vi "Login.vi"(8 "error in (no error) 3":errorcluster) -> (0 "error in (no error) 4":errorcluster, 3 "Enum":T2)   [LabVIEW 2021]
uses:
  Control/login_type.ctl
  Control/User_login_type.ctl
  Control/add_remove.ctl
  Template/Main_VI/Control/Ini.ctl
panel:
  in  "USER TYPE":T1 items=["Admin", "Operator"]
  out "element 3":string
  out "Array 2":string[](array[string])
  in  "PASSWORD":string
  in  "NAME":T1
  out "element 2":string
  in  "Remove user":bool
  out "Boolean 4":bool=TRUE
  out "Numeric":i32
  out "Boolean 3":bool=TRUE
  in  "Back Button":bool
  in  "Enum":T2
  in  "error in (no error) 2":errorcluster
  out "error out":errorcluster
  out "Result":bool
  out "element":string
  out "Ring - Menu 2":u16(ring)
  in  "error in (no error)":errorcluster
  out "array w/ subset deleted":string[](array[string])
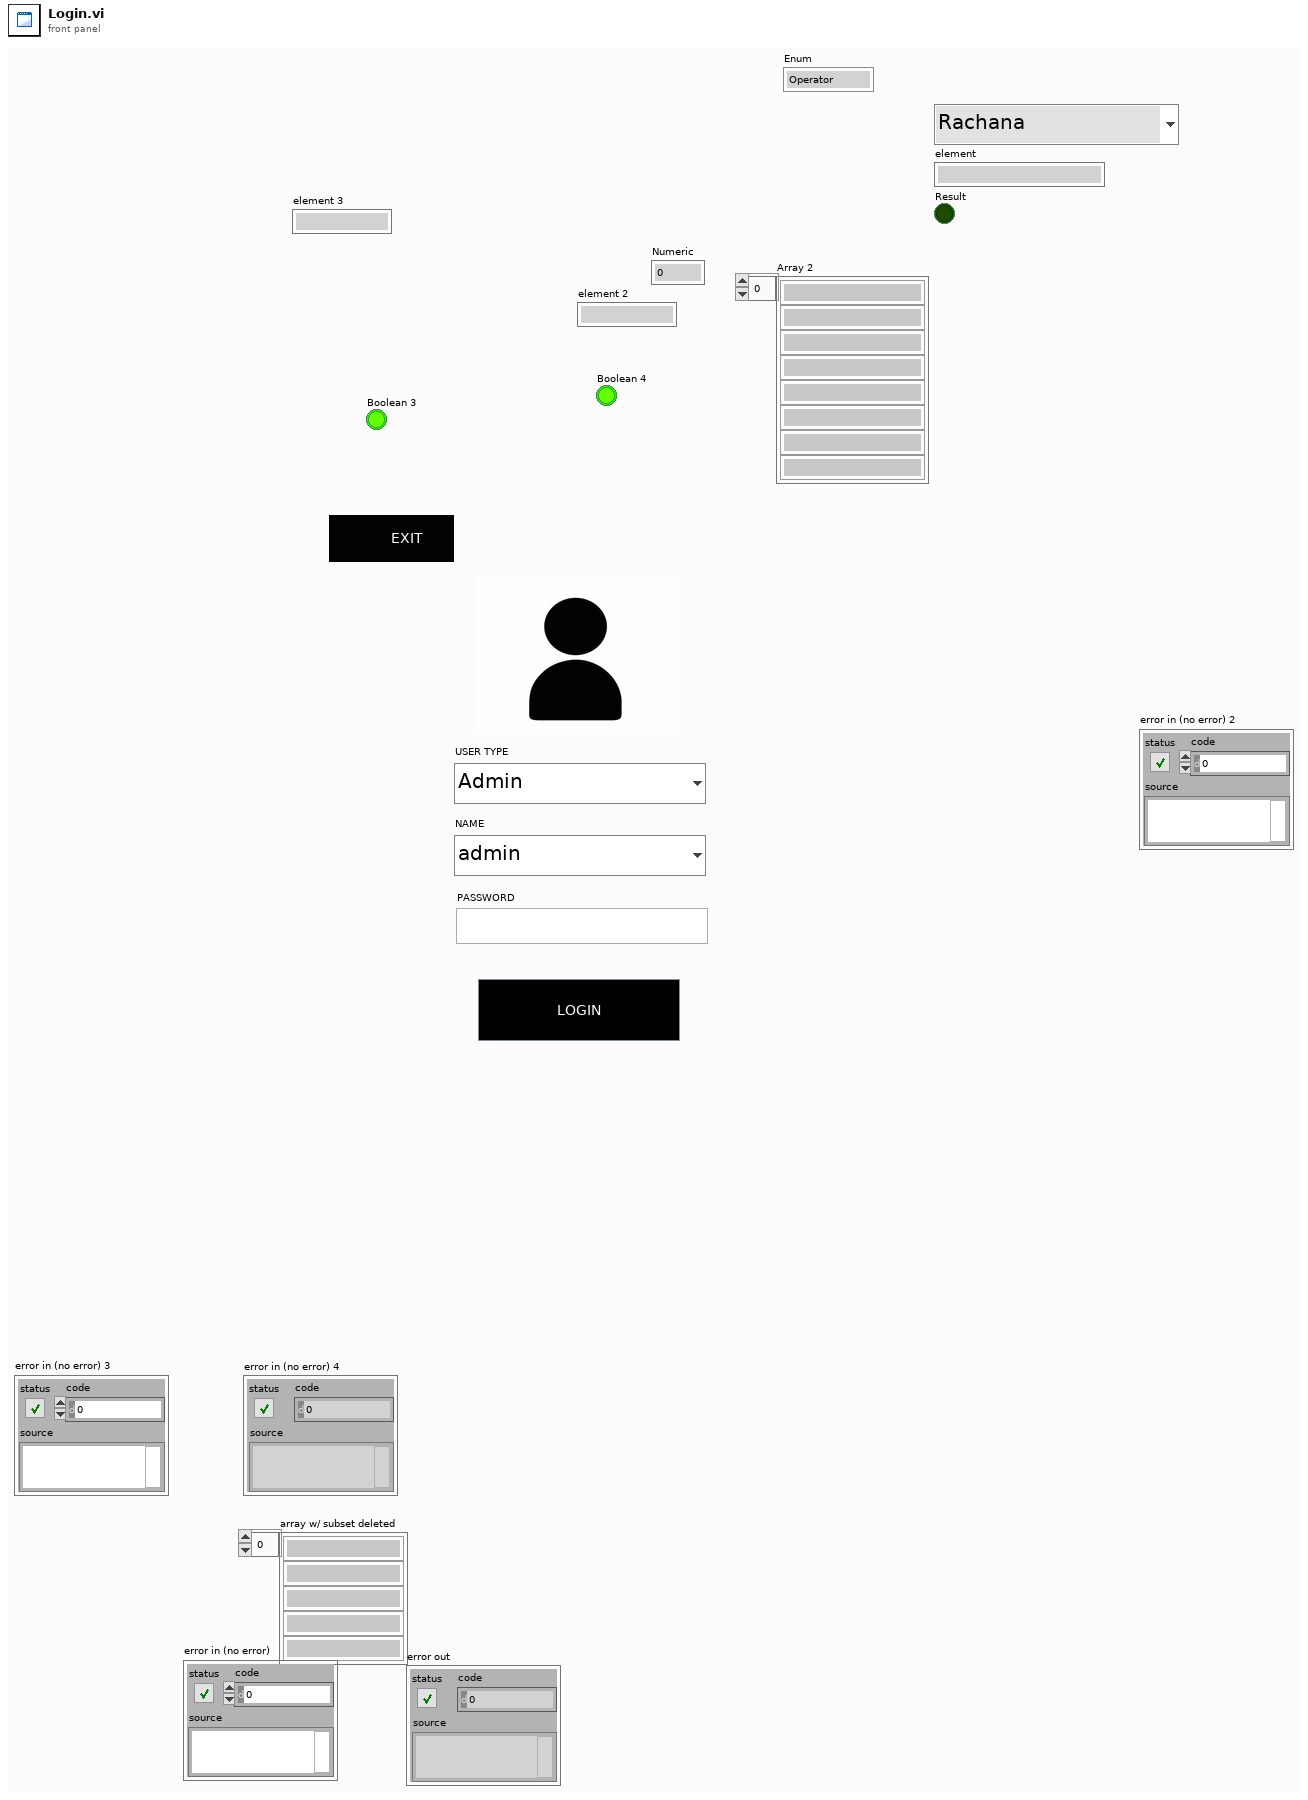
[diagram p1: front panel]
types:
  T1 = typedef "User_login_type.ctl" = u16
  T2 = typedef "login_type.ctl" = enum16{"Operator", "Admin"}
  T3 = typedef "add_remove.ctl" = enum16{"Enter", "add user", "remover user", "view user"}
  T4 = typedef "Ini.ctl" = enum16{"Write", "Read"}
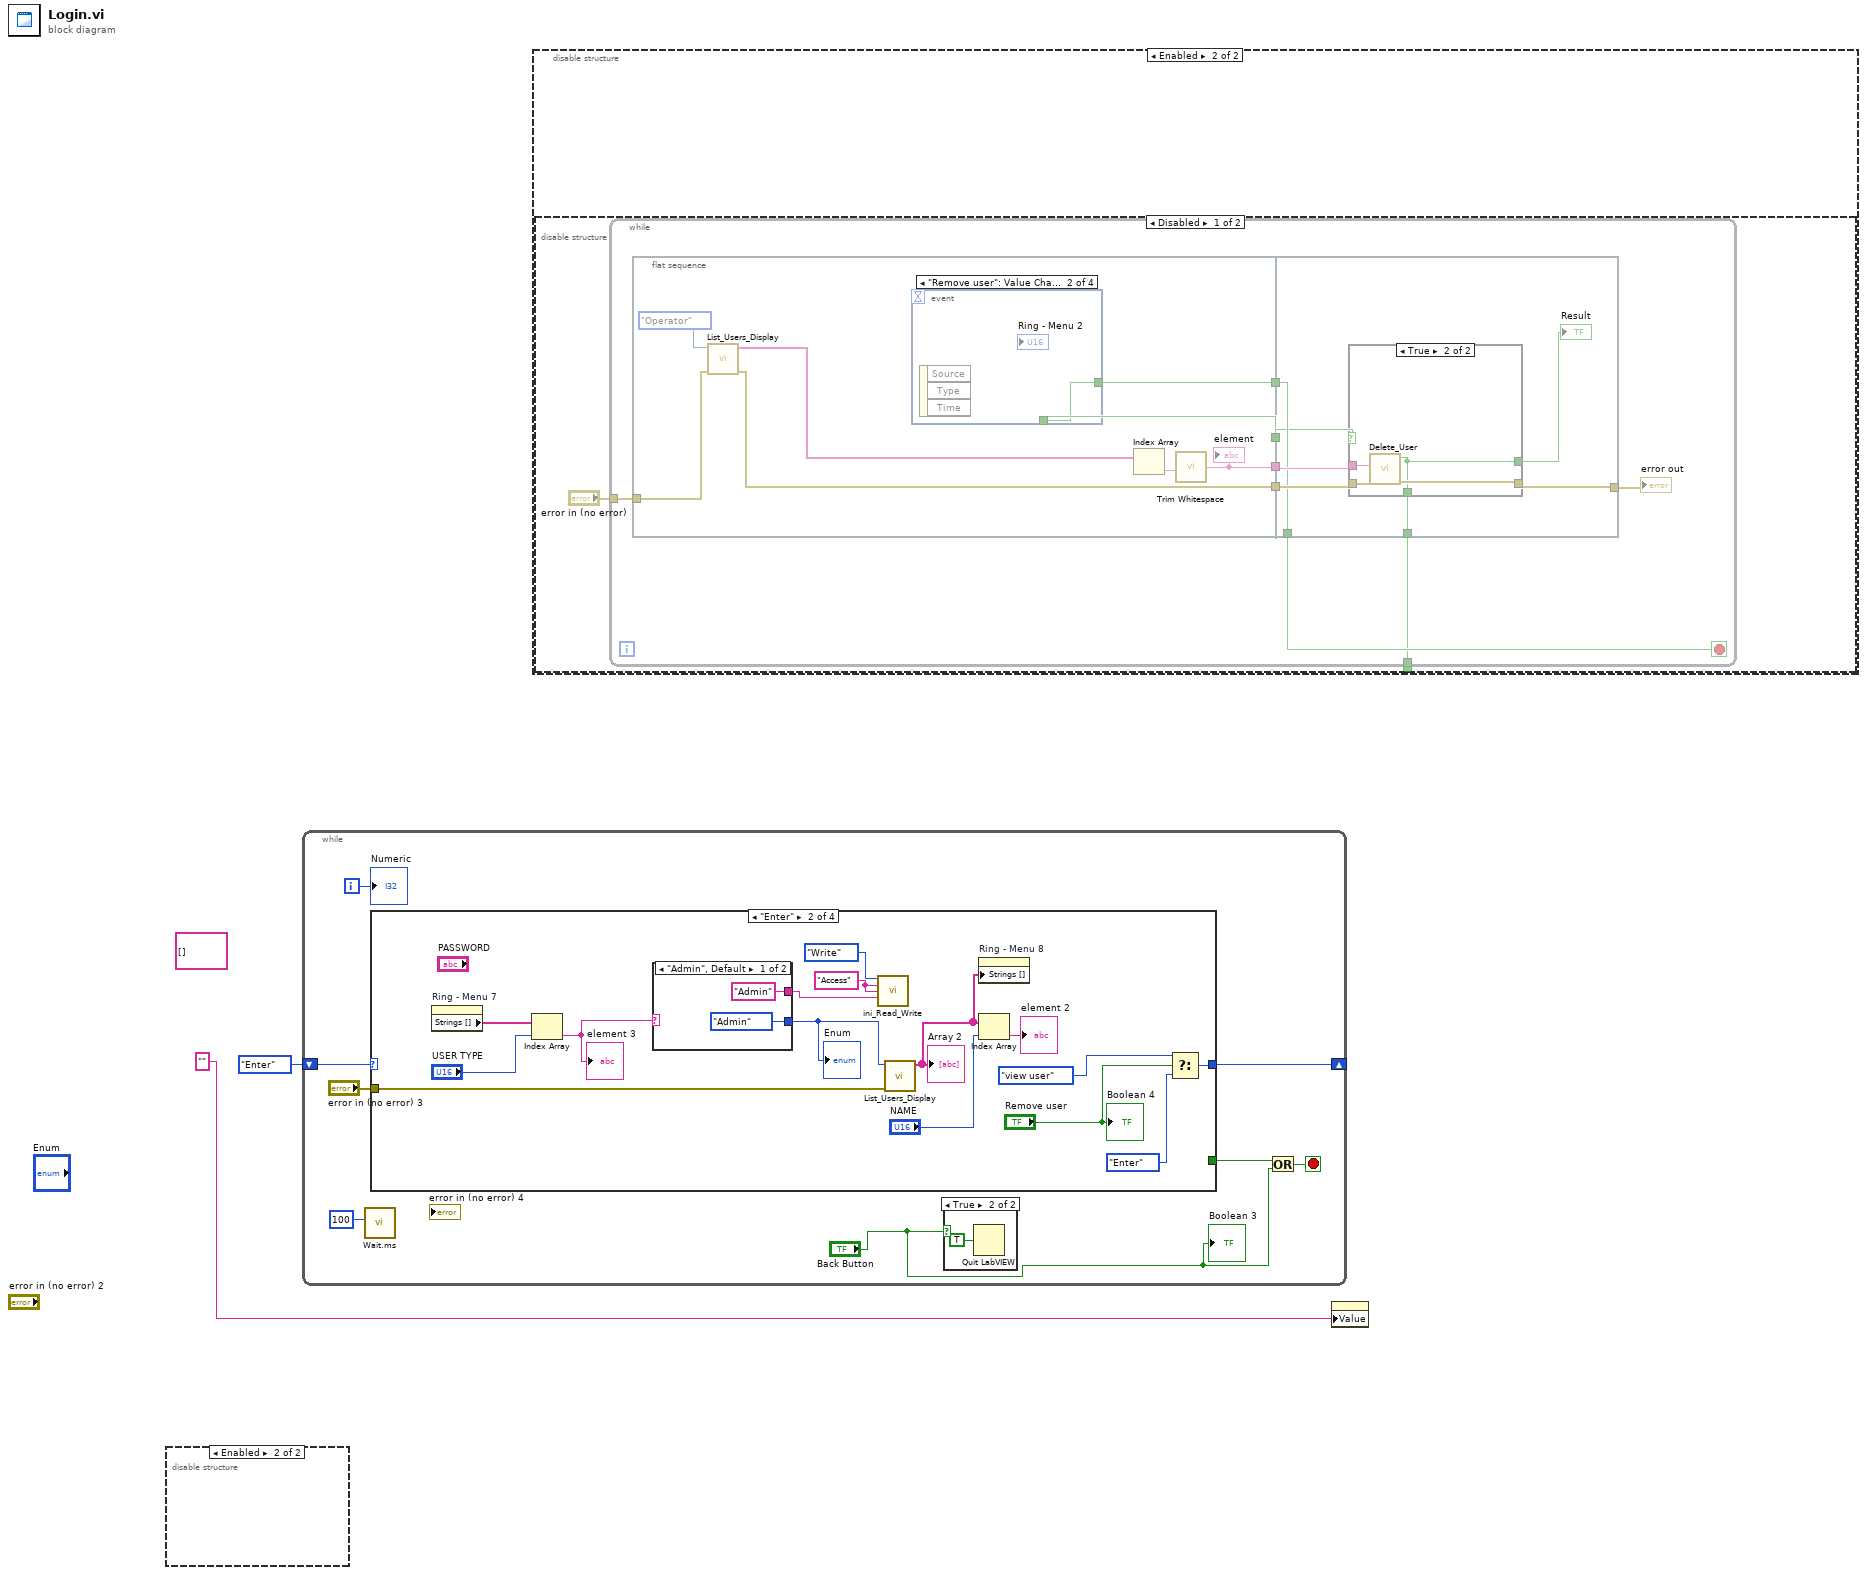
[diagram p0: block diagram]
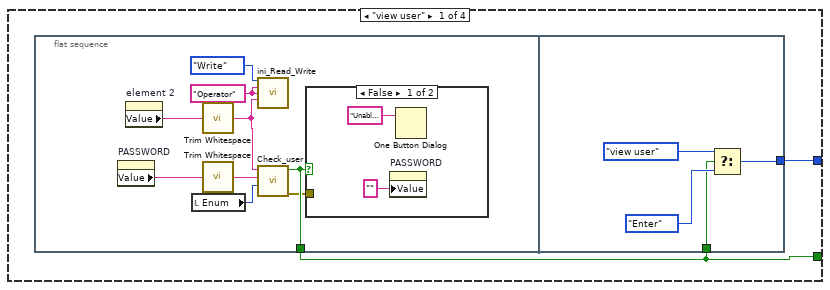
[diagram p3: hidden frame]
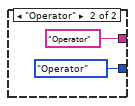
[diagram p5: hidden frame]
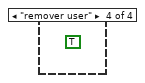
[diagram p7: hidden frame]
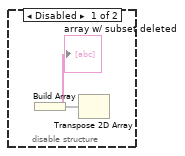
[diagram p9: hidden frame]
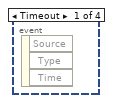
[diagram p10: hidden frame]
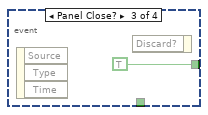
[diagram p11: hidden frame]
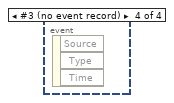
[diagram p12: hidden frame]
diagram:
  (unwired) string[][] [] ("Item Names")
  n1 = disable-structure shown="Enabled" {
    frame Disabled {
    }
    frame Enabled {
    }
  }
  n2 = while {
    shift-right: [w9] -> _
    shift-left: add_remove."Enter" -> [w10]
    i -> [w8]
    stop <- w4 stop-if-true
    n3 = call "Wait.ms.vi"("milliseconds to wait"=u32 100) -> ()  [unwired: 10 in, 1 out]
    n4 = case shown="\"Enter\"" w10 {
      tunnel: [w12 w33 _ _] -> w9
      tunnel: "error in (no error) 3" -> [_ w39 _ _]
      tunnel: [w13 _ _ _] -> w5
      frame "view user" {
        n5 = flat-sequence {
          tunnel: [w21] -> w13
          tunnel: w13 -> [w27]
          tunnel: [w25] -> w12
          frame #0 {
            w15 = "Operator" ("Write Section")
            n6 = property on="PASSWORD" class="Str"() -> ("Value"=w17:string)  [unwired: 2 in, 2 out]
            n7 = property on="element 2" class="Str"() -> ("Value"=w19:string)  [unwired: 2 in, 2 out]
            n8 = local read "Enum"() -> (w22:T2)
            n9 = call <vilib>:"Trim Whitespace.vi"("string"=w19) -> ("trimmed string"=w14:string)  [unwired: 1 in]
            n10 = call <vilib>:"Trim Whitespace.vi"("string"=w17) -> ("trimmed string"=w18:string)  [unwired: 1 in]
            n11 = call "ini_Read_Write.vi"(0:Ini."Write", "Write Section"=w15, "Write key"=w15, "Write"=w14) -> ()  [unwired: 10 in, 2 out]
            n12 = call "Check_user.vi"("Enum"=w22, "Password"=w18, "Name"=w14) -> ("error out"=w20:errorcluster, "Result"=w21:bool)  [unwired: 7 in]
            n13 = case shown="False" w21 {
              tunnel: w20 -> [_ _]
              frame False {
                n14 = property on="PASSWORD" class="Str"("Value"="" ("Password 3")) -> ()  [unwired: 2 in, 2 out]
                n15 = One Button Dialog(message="Unable to login Check ID and password") -> ()  [unwired: 1 in, 1 out]
              }
              frame True {
              }
            }
          }
          frame #1 {
            n16 = Select(t=add_remove."view user", s=w27, f=add_remove."Enter") -> (s? t:f=w25:T3)
          }
        }
      }
      frame "Enter" {
        w30 = "Access" ("Write")
        n17 = property on="Ring - Menu 7" class="Ring (strict)"() -> ("Strings []"=w43:string[])  [unwired: 2 in, 2 out]
        n18 = Index Array(array=w43, index="USER TYPE") -> (element=w41:string)
        "element 3" <- w41
        n19 = case shown="\"Admin\", Default" w41 {
          tunnel: [login_type."Admin" login_type."Operator"] -> w40
          tunnel: ["Admin" ("Write") "Operator" ("Write")] -> w29
          frame "Admin", Default {
          }
          frame "Operator" {
          }
        }
        "Enum" <- w40
        n20 = call "ini_Read_Write.vi"(0:Ini."Write", "Write Section"=w30, "Write key"=w30, "Write"=w29) -> ()  [unwired: 10 in, 2 out]
        n21 = call "List_Users_Display.vi"("error in (no error)"=w39, "Enum"=w40) -> ("Array"=w38:string[])  [unwired: 8 in, 1 out]
        "Array 2" <- w38
        n22 = property on="Ring - Menu 8" class="Ring (strict)"("Strings []"=w38) -> ()  [unwired: 2 in, 2 out]
        n23 = Index Array(array=w38, index="NAME") -> (element=→"element 2":string)
        n24 = Select(t=add_remove."view user", s="Remove user", f=add_remove."Enter") -> (s? t:f=w33:T3)
        "Boolean 4" <- "Remove user"
      }
      frame "add user" {
      }
      frame "remover user" {
        (unwired) TRUE
      }
    }
    n25 = case shown="True" "Back Button" {
      frame False {
      }
      frame True {
        n26 = Quit LabVIEW(quit? (T)=TRUE) -> ()
      }
    }
    n27 = Or(x=w5, y="Back Button") -> (x .or. y?=w4:bool)
    "Numeric" <- w8
    "Boolean 3" <- "Back Button"
  }
  n28 = disable-structure shown="Enabled" {
    frame Disabled {
      n29 = Build Array("array w/ subset deleted") -> (w48:void[])
      n30 = Transpose 2D Array(2D array=w48) -> (transposed array=w49:void[][])
    }
    frame Enabled {
      n31 = disable-structure shown="Disabled" {
        disable-tunnel: [w51 _] -> _
        frame Disabled {
          n32 = while {
            tunnel: "error in (no error)" -> [w58]
            tunnel: [w53] -> w51
            stop <- w55 stop-if-true
            n33 = flat-sequence {
              tunnel: [w67] -> w60
              tunnel: w58 -> [w64]
              tunnel: [w63] -> w59
              tunnel: [w66] -> w56
              tunnel: [w65] -> w54
              tunnel: w60 -> [w77]
              tunnel: w59 -> [w76]
              tunnel: [w75] -> w57
              tunnel: w56 -> [w74]
              tunnel: [w74] -> w55
              tunnel: w54 -> [w73]
              tunnel: [w71] -> w53
              frame #0 {
                n34 = call "List_Users_Display.vi"("error in (no error)"=w64, "Enum"=login_type."Operator") -> ("error out"=w63:errorcluster, "Array"=w61:string[])  [unwired: 8 in]
                n35 = event shown="[1] \"Remove user\": Value Change" {
                  selector: _ -> [_ _ _ _]
                  dyn-events: _ -> [_ _ _ _]
                  timeout: _ -> [_ _ _ _]
                  tunnel: [_ w69 TRUE _] -> w66
                  tunnel: [_ w69 _ _] -> w65
                  event Timeout {
                    n36 = event-data() -> ()  [unwired: 1 in, 3 out]
                  }
                  event "Remove user": Value Change {
                    n37 = event-data() -> ()  [unwired: 1 in, 3 out]
                  }
                  event Panel Close? {
                    n38 = event-data() -> ()  [unwired: 1 in, 3 out]
                    n39 = event-data() -> ()  [unwired: 2 in, 1 out]
                  }
                  event #3 (no event record) {
                    n40 = event-data() -> ()  [unwired: 1 in, 3 out]
                  }
                }
                n41 = Index Array(array=w61) -> (element=w68:string)  [unwired: 1 in]
                n42 = call <vilib>:"Trim Whitespace.vi"("string"=w68) -> ("trimmed string"=w67:string)  [unwired: 1 in]
                "element" <- w67
              }
              frame #1 {
                n43 = case shown="True" w73 {
                  tunnel: w77 -> [_ w82]
                  tunnel: [_ w79] -> w72
                  tunnel: w76 -> [w78 w81]
                  tunnel: [w78 w80] -> w75
                  tunnel: [_ w79] -> w71
                  frame False {
                  }
                  frame True {
                    n44 = call "Delete_User.vi"("error in (no error)"=w81, "Name"=w82) -> ("error out"=w80:errorcluster, "Result"=w79:bool)  [unwired: 8 in]
                  }
                }
                "Result" <- w72
              }
            }
            "error out" <- w57
          }
        }
        frame Enabled {
        }
      }
    }
  }
  n45 = property on="PASSWORD" class="Str"("Value"="" ("Name 3")) -> ()  [unwired: 2 in, 2 out]
